vi "Process Packet.vi"(8 "error in (no error)":errorcluster, 10 "Incoming Packet":refnum<class "ControlPacket.lvclass">, 11 "Session in":refnum<class "Session.lvclass">) -> (0 "error out":errorcluster, 3 "Session out":refnum<class "Session.lvclass">)   [LabVIEW 2013, in "MQTT Base.lvlib" / "Session.lvclass"]
uses:
  Session.lvclass
  <vilib>/LabVIEW Open Source Project/MQTT Control Packets/Control Packets/ControlPacket/ControlPacket.lvclass
  Base Class/Request -- cluster.ctl
  Base Class/Response -- cluster.ctl
  Session.lvclass/Session.ctl
  Base Class/MQTT_Base.lvclass
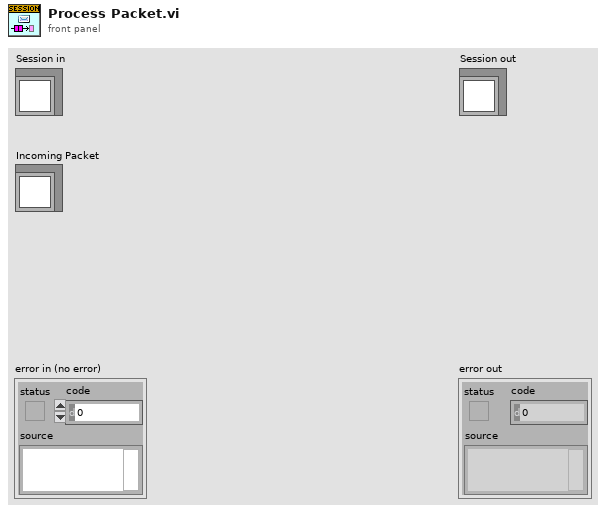
[diagram p1: front panel]
types:
  T1 = typedef "MQTT Base.lvlib/MQTT_Base.lvclass/Request -- cluster.ctl" = cluster{"Packet":refnum<class "ControlPacket.lvclass">, "SessionMailbox":refnum<queue>}
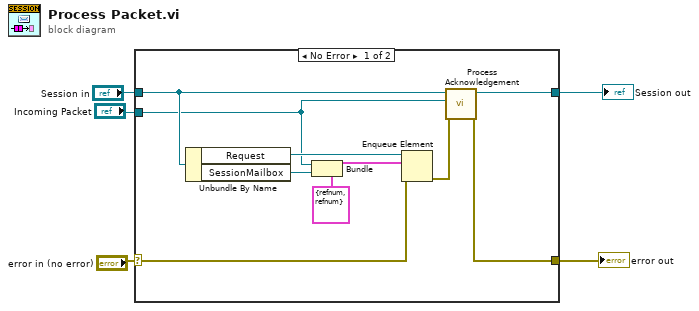
[diagram p0: block diagram]
diagram:
  n1 = case shown="No Error" "error in (no error)" {
    selector: "error in (no error)" -> [w9 w17]
    tunnel: [w7 w17] -> w1
    tunnel: [w15 w16] -> w2
    tunnel: "Session in" -> [w10 w16]
    tunnel: "Incoming Packet" -> [w6 _]
    frame No Error {
      n2 = Unbundle By Name(w10) -> ("Request"=w11:refnum<queue>, "SessionMailbox"=w12:refnum<queue>)
      n3 = Bundle(cluster=T1 {"Packet"=refnum, "SessionMailbox"=refnum} ("Request"), "Packet"=w6, "SessionMailbox"=w12) -> (w13:T1)
      n4 = Enqueue Element(queue=w11, element=w13, error in (no error)=w9) -> (error out=w8:errorcluster)  [unwired: 1 in, 2 out]
      n5 = call "Process Acknowledgement.vi"("error in (no error)"=w8, "Incoming Packet"=w6, "Session in"=w10) -> ("error out"=w7:errorcluster, "Session out"=w15:refnum<class "Session.lvclass">)  [unwired: 7 in]
    }
    frame Error {
    }
  }
  "error out" <- w1
  "Session out" <- w2
